vi "ElevatorSim_UpdateX.vi"(8 "dT_Seconds":dbl=0.02, 9 "U":T4, 10 "current_xHat":T4, 11 "ELEVATOR_SIM":T1={"LinearSystemSim"={"m_Plant"={"m_A"=[], "m_B"=[], "m_C"=[], "m_D"=[], "States"=0, "Inputs"=0, "Outputs"=0}, "m_X"=[], "m_Y"=[], "m_U"=[], "MeasureStdDev"=[]}, "GearBox"={"nominalVoltage_Volts"=0.0, "StallTorque_NM"=0.0, "StallCurrent_Amps"=0.0, "FreeCurrent_Amps"=0.0, "FreeSpeed_RadPerSec"=0.0, "R_Ohms"=0.0, "KvINV_RadPerSecPerVolt"=0.0, "Kt_NMPerAmp"=0.0, "L_H"=0.0, "Jr_KgM2"=0.0}, "Gearing"=0.0, "DrumRadius_M"=0.0, "MinHeight_M"=0.0, "MaxHeight_M"=0.0, "CarriageMass_Kg"=0.0, "SimulateGravity"=TRUE} {"GearBox"."Jr_KgM2" format="%13.5p"; "GearBox"."L_H" format="%13.5p"; "GearBox"."Kt_NMPerAmp" format="%13.5p"; "GearBox"."KvINV_RadPerSecPerVolt" format="%13.5p"; "GearBox"."R_Ohms" format="%13.5p"; "GearBox"."FreeSpeed_RadPerSec" format="%13.5p"; "GearBox"."FreeCurrent_Amps" format="%13.5p"; "GearBox"."StallCurrent_Amps" format="%13.5p"; "GearBox"."StallTorque_NM" format="%13.5p"; "GearBox"."nominalVoltage_Volts" format="%13.5p"}) -> (0 "Error":bool, 3 "updated_xHat":T4)   [LabVIEW 2019, in "Trajectory_Library.lvlib"]
doc: "Updates the state of the elevator.\n \nInputs:\n - ElevatorSim -- Data cluster\n - currentXhat -- The current state estimate.\n - u -- The system inputs (voltage).\n - dtSeconds -- he time difference between controller updates.\n\nOutputs:\n - OutElevatorSim -- Updated data cluster\n - Error -- If TRUE, an error occured."
uses:
  Trajectory_Library.lvlib
  <vilib>/Analysis/Matrix/Datatypes/RealMatrix.ctl
  <vilib>/Analysis/Matrix/NI_Matrix.lvlib
  TypeDef/LINEAR_SYSTEM.ctl
  TypeDef/LINEAR_SYSTEM_SIM.ctl
  TypeDef/DCMOTOR.CTL
  TypeDef/ELEVATOR_SIM.ctl
panel:
  # "<States, 1>"
  # "<Outputs, 1>"
  # "<Inputs, 1>"
  # "<Outputs, 1>"
  # "<States,States>"
  # "<States,Inputs>"
  # "<Outputs,States>"
  # "<Outputs,Inputs>"
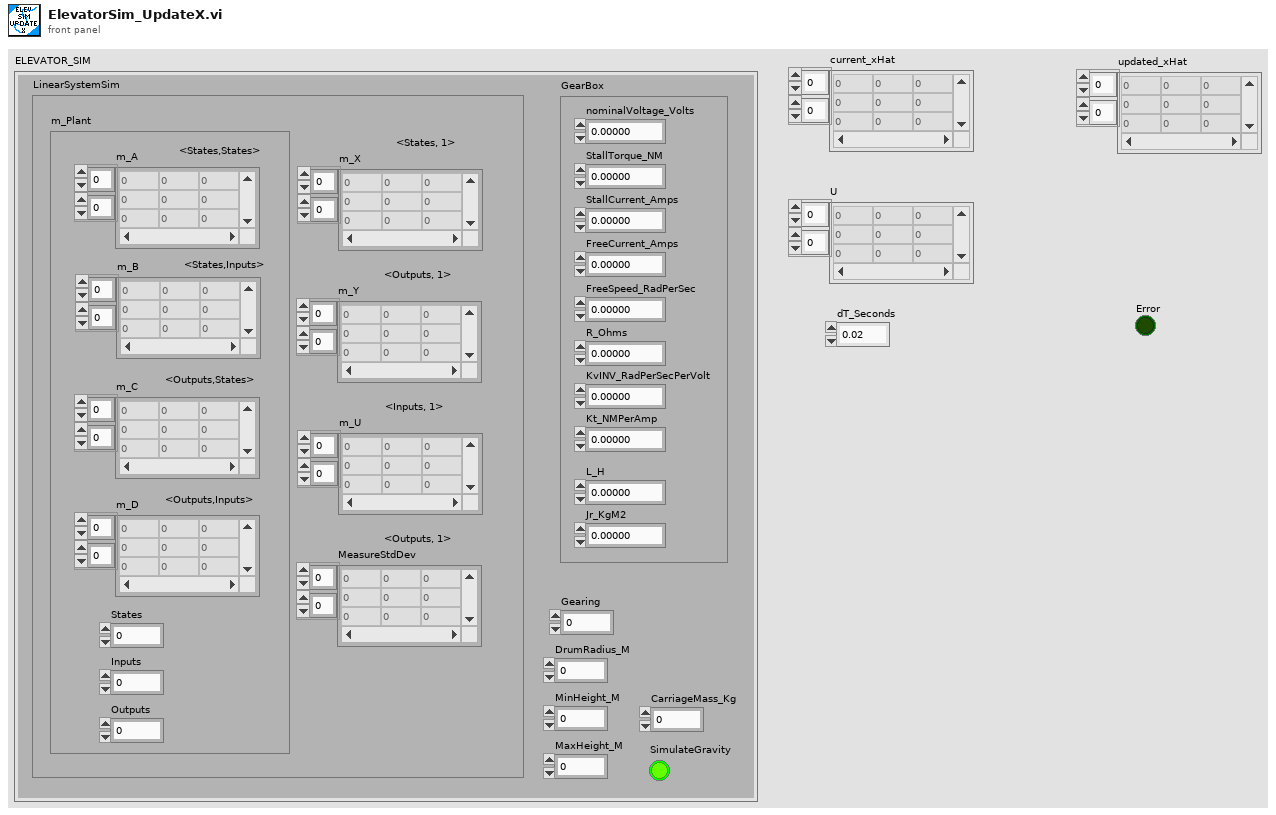
[diagram p1: front panel]
types:
  T1 = typedef "Trajectory_Library.lvlib/ELEVATOR_SIM.ctl" = cluster{"LinearSystemSim":T2, "GearBox":T5, "Gearing":dbl, "DrumRadius_M":dbl, "MinHeight_M":dbl, "MaxHeight_M":dbl, "CarriageMass_Kg":dbl, "SimulateGravity":bool}
  T2 = typedef "Trajectory_Library.lvlib/LINEAR_SYSTEM_SIM.ctl" = cluster{"m_Plant":T3, "m_X":T4, "m_Y":T4, "m_U":T4, "MeasureStdDev":T4}
  T3 = typedef "Trajectory_Library.lvlib/LINEAR_SYSTEM.ctl" = cluster{"m_A":T4, "m_B":T4, "m_C":T4, "m_D":T4, "States":i32, "Inputs":i32, "Outputs":i32}
  T4 = typedef "NI_Matrix.lvlib/RealMatrix.ctl" = dbl[][]
  T5 = typedef "Trajectory_Library.lvlib/DCMOTOR.CTL" = cluster{"nominalVoltage_Volts":dbl, "StallTorque_NM":dbl, "StallCurrent_Amps":dbl, "FreeCurrent_Amps":dbl, "FreeSpeed_RadPerSec":dbl, "R_Ohms":dbl, "KvINV_RadPerSecPerVolt":dbl, "Kt_NMPerAmp":dbl, "L_H":dbl, "Jr_KgM2":dbl}
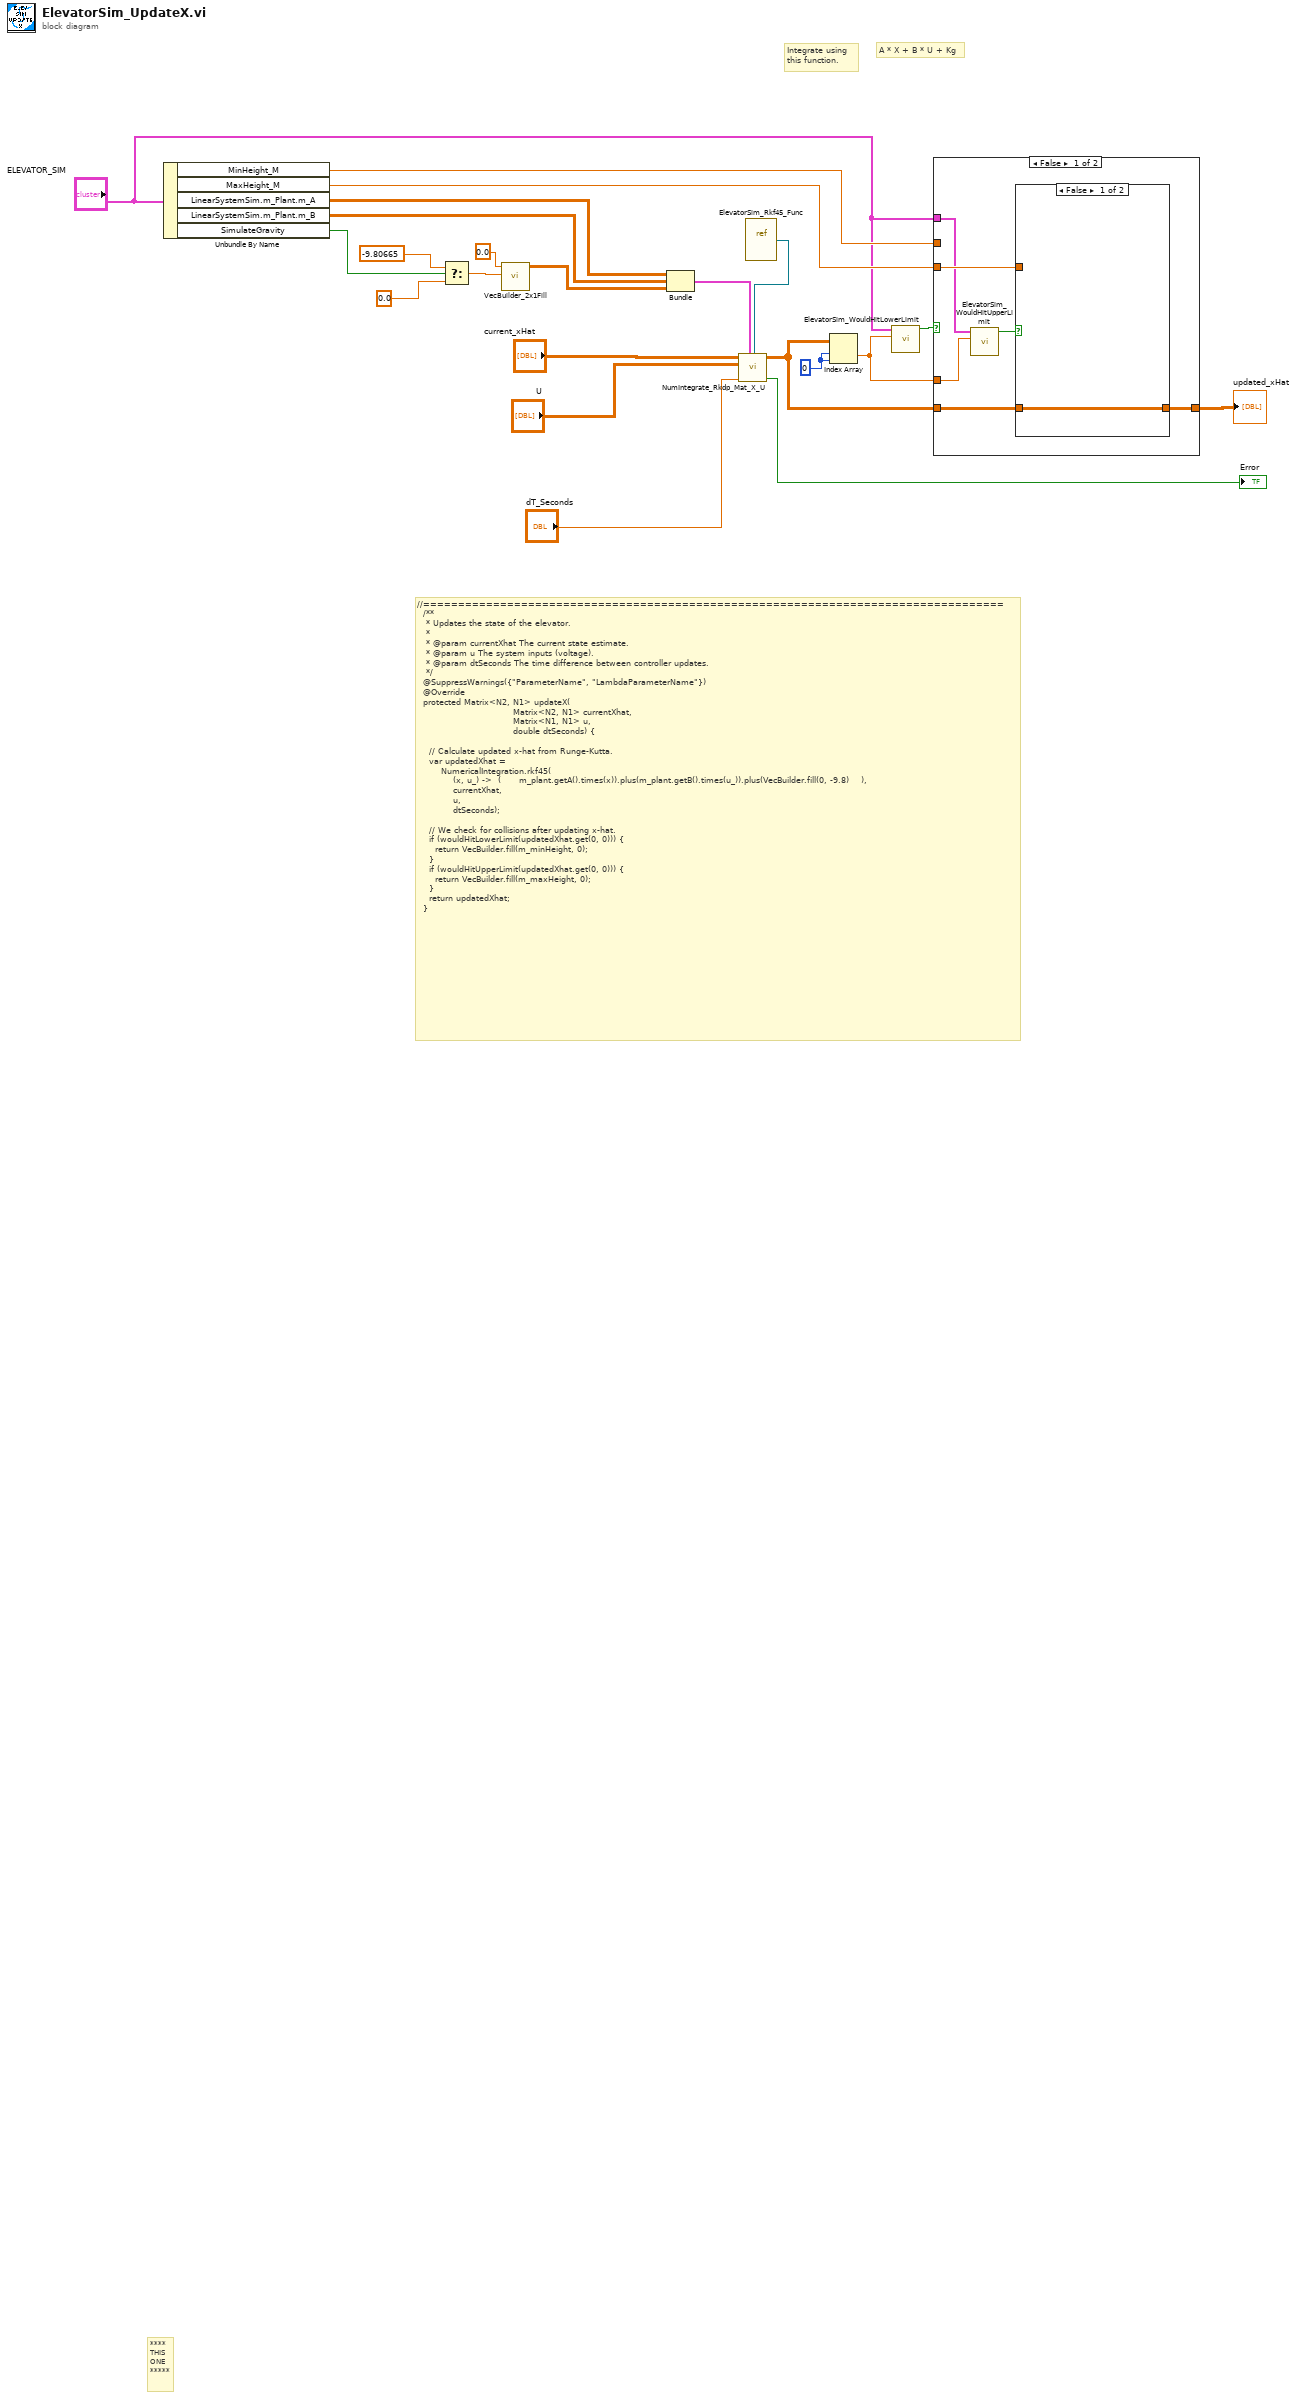
[diagram p0: block diagram]
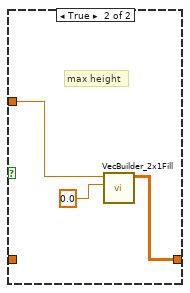
[diagram p2: hidden frame]
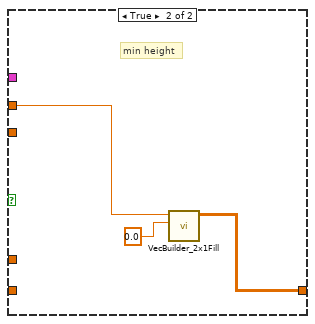
[diagram p3: hidden frame]
diagram:
  w18 = 0 ("index (row)")
  # "Integrate using\nthis function."
  # "A * X + B * U + Kg"
  # "//===================================================================================\n  /**\n   * Updates the state of the elevator.\n   *\n   * @param currentXhat The current state estimate.\n   * @param u The system inputs (voltage).\n   * @param dtSeconds The time difference between controller updates.\n   */\n  @SuppressWarnings({\"ParameterName\", \"LambdaParameterName\"})\n  @Override\n  protected Matrix<N2, N1> updateX(\n                                Matrix<N2, N1> currentXhat, \n                                Matrix<N1, N1> u, \n                                double dtSeconds) {\n\n    // Calculate updated x-hat from Runge-Kutta.\n    var updatedXhat =\n        NumericalIntegration.rkf45(\n            (x, u_) ->  (      m_plant.getA().times(x)).plus(m_plant.getB().times(u_)).plus(VecBuilder.fill(0, -9.8)    ),\n            currentXhat,\n            u,\n            dtSeconds);\n\n    // We check for collisions after updating x-hat.\n    if (wouldHitLowerLimit(updatedXhat.get(0, 0))) {\n      return VecBuilder.fill(m_minHeight, 0);\n    }\n    if (wouldHitUpperLimit(updatedXhat.get(0, 0))) {\n      return VecBuilder.fill(m_maxHeight, 0);\n    }\n    return updatedXhat;\n  }"
  # "****\nTHIS\nONE\n*****"
  n1 = Unbundle By Name("ELEVATOR_SIM") -> ("MinHeight_M"=w12:dbl, "MaxHeight_M"=w17:dbl, "LinearSystemSim.m_Plant.m_A"=w10:T4, "LinearSystemSim.m_Plant.m_B"=w9:T4, "SimulateGravity"=w3:bool)
  n2 = Select(t=-9.80665 ("R1"), s=w3, f=0.0) -> (s? t:f=w4:dbl)
  n3 = call "VecBuilder_2x1Fill.vi"("R1"=w4, "R0"=0.0) -> ("output matrix"=w8:T4)  [unwired: 9 in]
  n4 = Bundle("m_A"=w10, "m_B"=w9, "output matrix"=w8) -> (w7:cluster{"m_A":T4, "m_B":T4, "output matrix":T4})  [unwired: 1 in]
  n5 = vi-ref "ElevatorSim_Rkf45_Func.vi"() -> (w6:refnum<vi>)
  n6 = call "NumIntegrate_Rkdp_Mat_X_U.vi"("Func_X_U_Extra"=w6, "PassedData"=w7, "dT_Seconds"="dT_Seconds", "U"="U", "X"="current_xHat") -> ("Error"=→"Error":bool, "Return X"=w16:T4)  [unwired: 4 in, 1 out]
  n7 = Index Array(array=w16, index (row)=w18, index (col)=w18) -> (element=w13:dbl)
  n8 = call "ElevatorSim_WouldHitLowerLimit.vi"("ElevHeight_Meters"=w13, "ElevatorSim"="ELEVATOR_SIM") -> ("WouldHitLowLimit"=w14:bool)  [unwired: 9 in]
  n9 = case shown="False" w14 {
    tunnel: w17 -> [w24 _]
    tunnel: w16 -> [w28 _]
    tunnel: [w27 w33] -> w15
    tunnel: w13 -> [w25 _]
    tunnel: w12 -> [_ w34]
    tunnel: "ELEVATOR_SIM" -> [w23 _]
    frame False {
      n10 = call "ElevatorSim_WouldHitUpperLimit.vi"("Height_Meters"=w25, "ElevatorSim"=w23) -> ("Would Hit Upper LImit"=w26:bool)  [unwired: 9 in]
      n11 = case shown="False" w26 {
        tunnel: w28 -> [w29 _]
        tunnel: [w29 w30] -> w27
        tunnel: w24 -> [_ w31]
        frame False {
        }
        frame True {
          # "max height"
          n12 = call "VecBuilder_2x1Fill.vi"("R1"=0.0, "R0"=w31) -> ("output matrix"=w30:T4)  [unwired: 9 in]
        }
      }
    }
    frame True {
      # "min height"
      n13 = call "VecBuilder_2x1Fill.vi"("R1"=0.0, "R0"=w34) -> ("output matrix"=w33:T4)  [unwired: 9 in]
    }
  }
  "updated_xHat" <- w15
